vi "AnotherOne.vi"() -> ()   [LabVIEW 2016]
uses:
  <vilib>/DAQmx/write.llb/DAQmx Write (Digital Bool 1Line 1Point).vi
  <vilib>/DAQmx/read.llb/DAQmx Read (Digital Bool 1Line 1Point).vi
  <vilib>/DAQmx/create/channels.llb/DAQmx Create Channel (DI-Digital Input).vi
  <vilib>/DAQmx/create/channels.llb/DAQmx Create Channel (DO-Digital Output).vi
  <vilib>/DAQmx/miscellaneous.llb/DAQmx Fill In Error Info.vi
panel:
  out "Start Button":bool
  out "Stop Button":bool
  out "Bottom Thing":bool
  out "Bottom Solenoid":bool
  in  "Chain Motor":bool
  in  "Sort Solenoid":bool
  in  "Rotary":bool
  in  "Belt motor":bool
  in  "Reject Solenoid":bool
  out "Assembled":bool
  out "Bottom Metal":bool
  out "Dropper Thing":bool
  out "Top Solenoid":bool
  out "Top Thing":bool
  out "Top Metal":bool
  in  "stop":bool
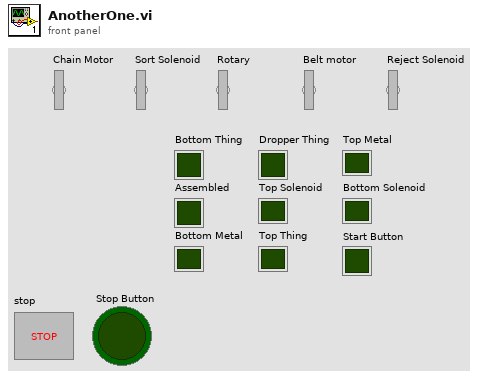
[diagram p1: front panel]
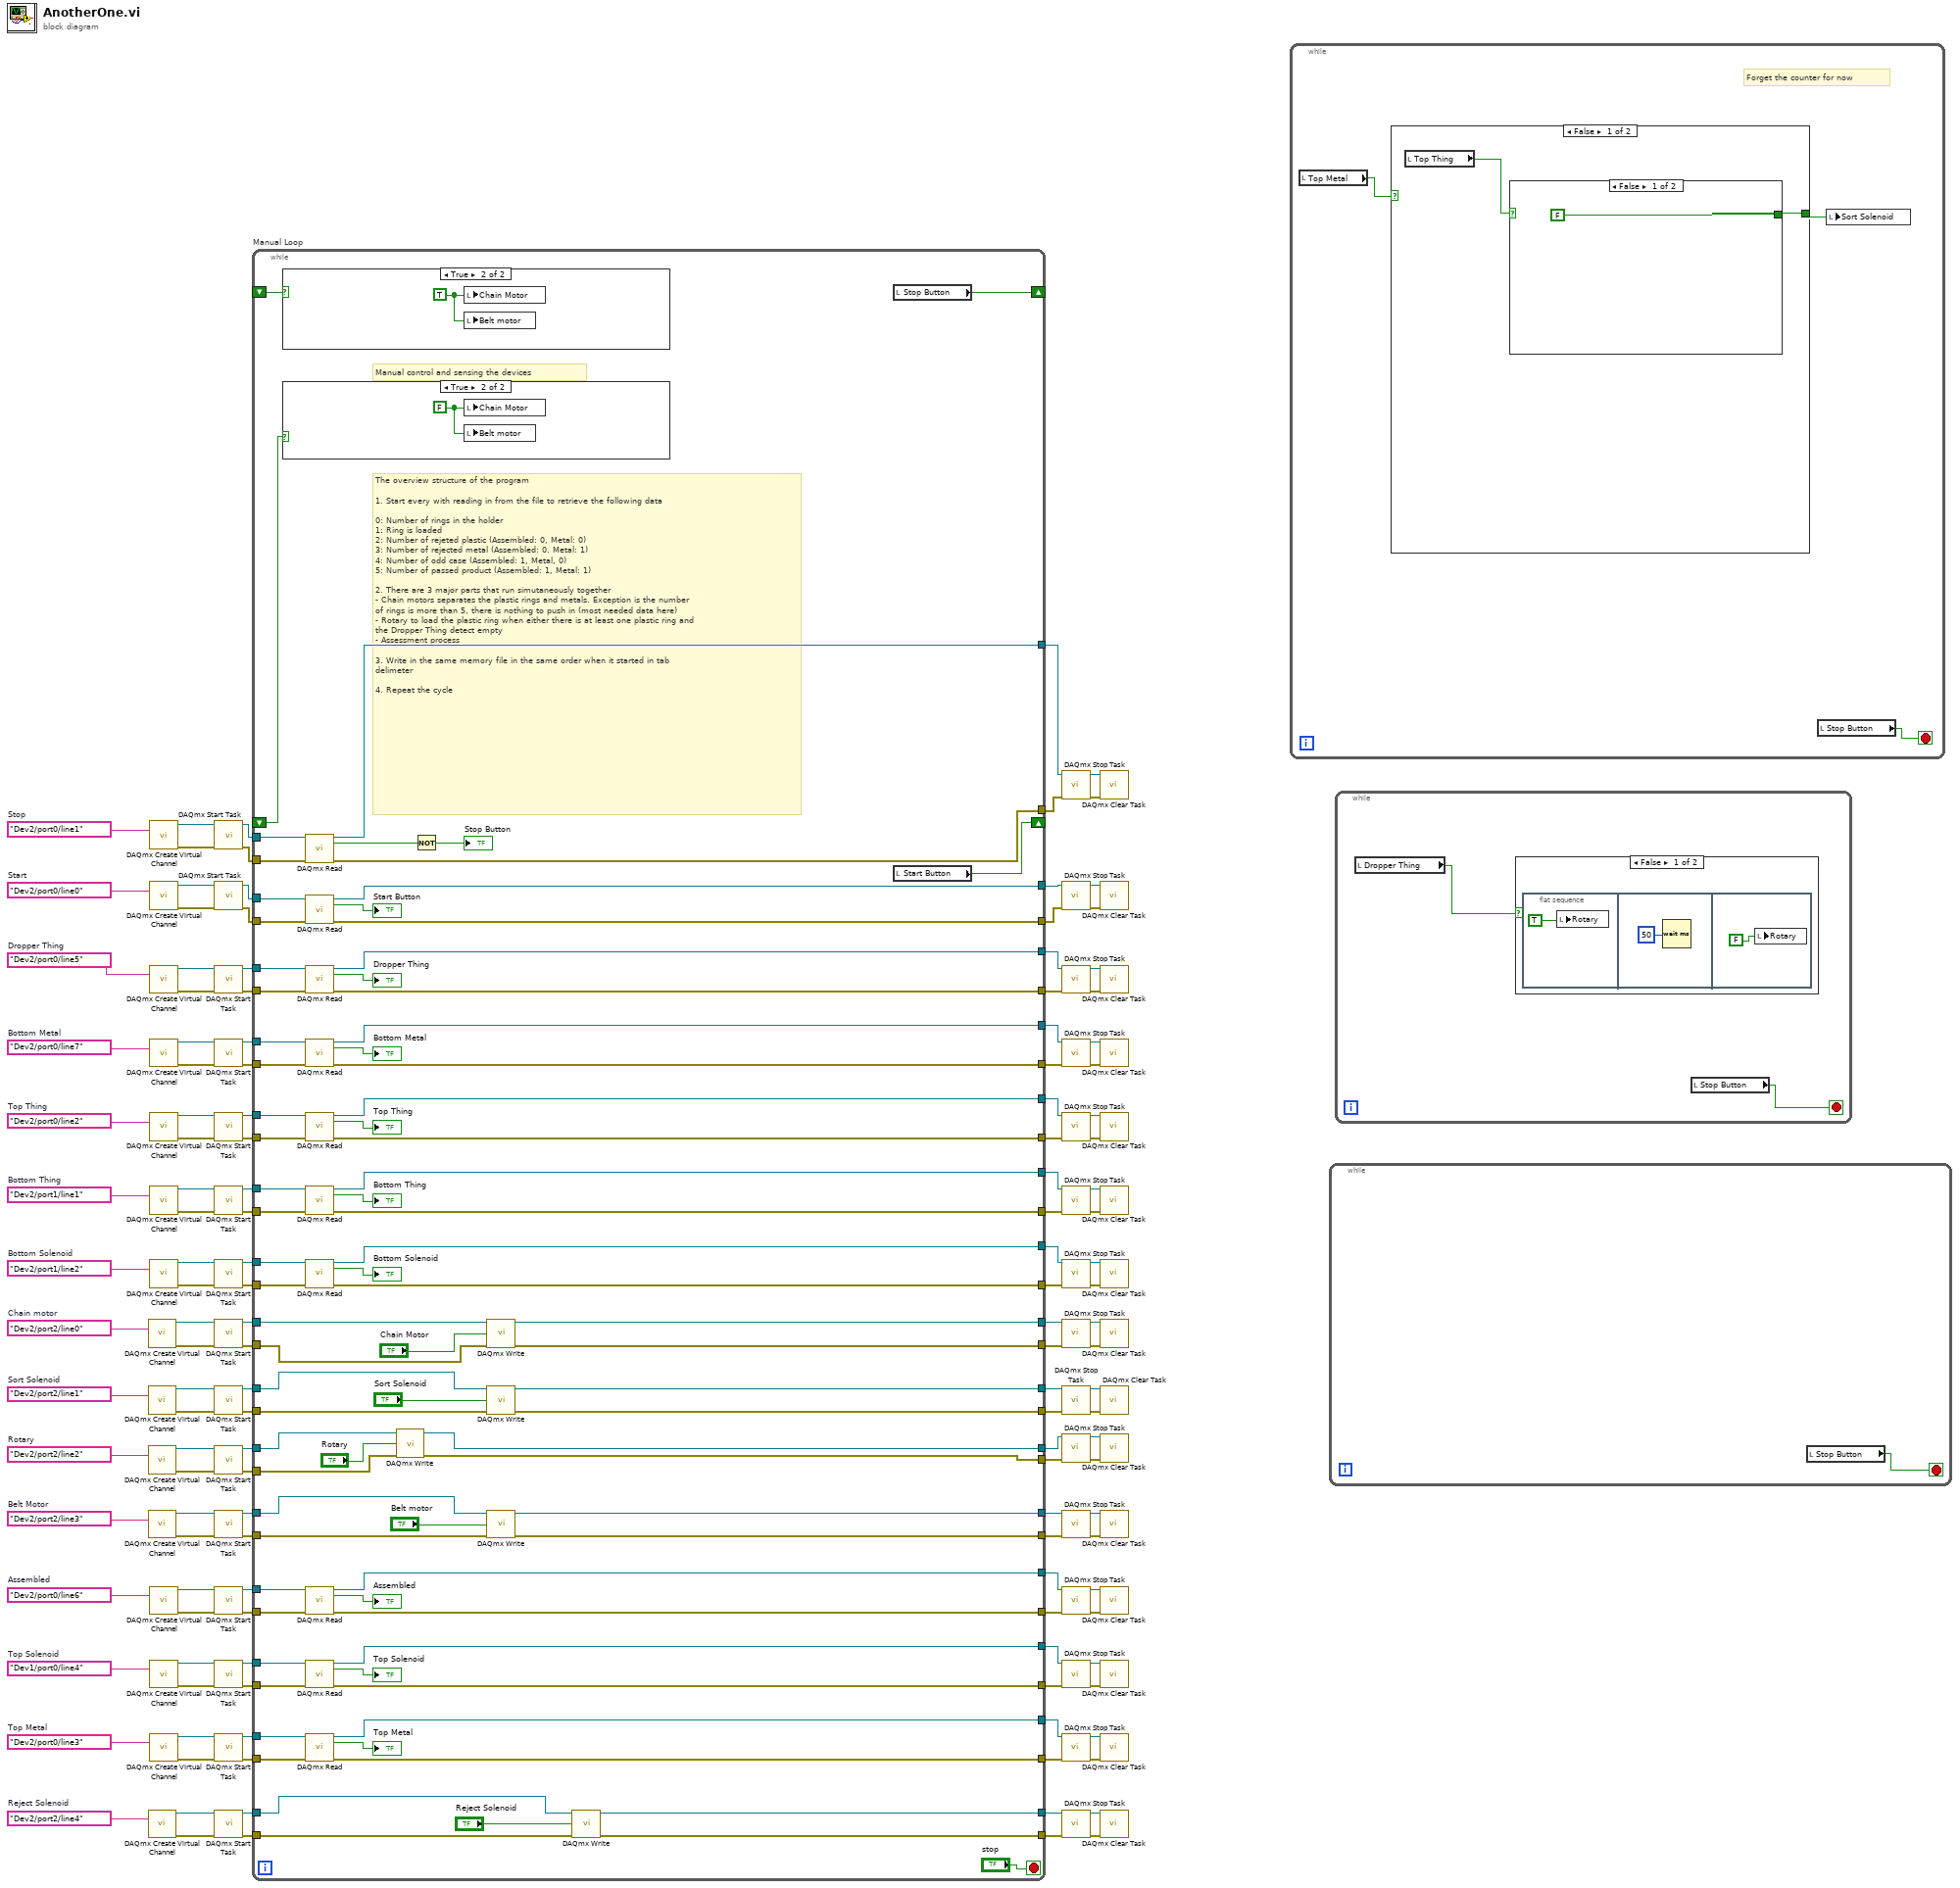
[diagram p0: block diagram]
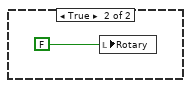
[diagram p2: hidden frame]
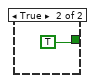
[diagram p3: hidden frame]
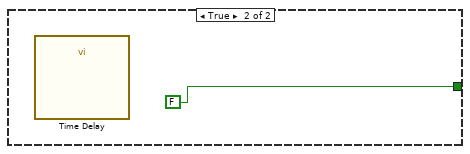
[diagram p4: hidden frame]
diagram:
  w95 = tag "Dev2/port1/line2"  # Bottom Solenoid
  w96 = tag "Dev2/port1/line1"  # Bottom Thing
  w101 = tag "Dev2/port0/line6"  # Assembled
  w102 = tag "Dev2/port0/line7"  # Bottom Metal
  w107 = tag "Dev2/port0/line5"  # Dropper Thing
  w108 = tag "Dev1/port0/line4"  # Top Solenoid
  w113 = tag "Dev2/port0/line3"  # Top Metal
  w114 = tag "Dev2/port0/line2"  # Top Thing
  w117 = tag "Dev2/port2/line4"  # Reject Solenoid
  w122 = tag "Dev2/port2/line3"  # Belt Motor
  w123 = tag "Dev2/port2/line2"  # Rotary
  w132 = tag "Dev2/port2/line1"  # Sort Solenoid
  w133 = tag "Dev2/port2/line0"  # Chain motor
  w134 = tag "Dev2/port0/line1"  # Stop
  w135 = tag "Dev2/port0/line0"  # Start
  n1 = call-poly <vilib>:"DAQmx Create Virtual Channel.vi"("lines"=w133) -> ("task out"=w127:refnum<k21>, "error out"=w126:errorcluster)  [unwired: 13 in]
  n2 = call-poly <vilib>:"DAQmx Create Virtual Channel.vi"("lines"=w132) -> ("task out"=w125:refnum<k21>, "error out"=w124:errorcluster)  [unwired: 13 in]
  n3 = call-poly <vilib>:"DAQmx Create Virtual Channel.vi"("lines"=w123) -> ("task out"=w121:refnum<k21>, "error out"=w120:errorcluster)  [unwired: 13 in]
  n4 = call-poly <vilib>:"DAQmx Create Virtual Channel.vi"("lines"=w122) -> ("task out"=w119:refnum<k21>, "error out"=w118:errorcluster)  [unwired: 13 in]
  n5 = call-poly <vilib>:"DAQmx Create Virtual Channel.vi"("lines"=w117) -> ("task out"=w116:refnum<k21>, "error out"=w115:errorcluster)  [unwired: 13 in]
  n6 = call-poly <vilib>:"DAQmx Create Virtual Channel.vi"("lines"=w134) -> ("task out"=w129:refnum<k21>, "error out"=w128:errorcluster)  [unwired: 13 in]
  n7 = call-poly <vilib>:"DAQmx Create Virtual Channel.vi"("lines"=w135) -> ("task out"=w130:refnum<k21>, "error out"=w131:errorcluster)  [unwired: 13 in]
  n8 = call-poly <vilib>:"DAQmx Create Virtual Channel.vi"("lines"=w107) -> ("task out"=w104:refnum<k21>, "error out"=w103:errorcluster)  [unwired: 13 in]
  n9 = call-poly <vilib>:"DAQmx Create Virtual Channel.vi"("lines"=w102) -> ("task out"=w99:refnum<k21>, "error out"=w100:errorcluster)  [unwired: 13 in]
  n10 = call-poly <vilib>:"DAQmx Create Virtual Channel.vi"("lines"=w114) -> ("task out"=w111:refnum<k21>, "error out"=w112:errorcluster)  [unwired: 13 in]
  n11 = call-poly <vilib>:"DAQmx Create Virtual Channel.vi"("lines"=w96) -> ("task out"=w93:refnum<k21>, "error out"=w94:errorcluster)  [unwired: 13 in]
  n12 = call-poly <vilib>:"DAQmx Create Virtual Channel.vi"("lines"=w95) -> ("task out"=w92:refnum<k21>, "error out"=w91:errorcluster)  [unwired: 13 in]
  n13 = call-poly <vilib>:"DAQmx Create Virtual Channel.vi"("lines"=w101) -> ("task out"=w98:refnum<k21>, "error out"=w97:errorcluster)  [unwired: 13 in]
  n14 = call-poly <vilib>:"DAQmx Create Virtual Channel.vi"("lines"=w108) -> ("task out"=w105:refnum<k21>, "error out"=w106:errorcluster)  [unwired: 13 in]
  n15 = call-poly <vilib>:"DAQmx Create Virtual Channel.vi"("lines"=w113) -> ("task out"=w110:refnum<k21>, "error out"=w109:errorcluster)  [unwired: 13 in]
  n16 = call <vilib>:"DAQmx Start Task.vi"("task/channels in"=w129, "error in"=w128) -> ("task out"=w88:refnum<k21>, "error out"=w87:errorcluster)  [unwired: 12 in]
  n17 = call <vilib>:"DAQmx Start Task.vi"("task/channels in"=w130, "error in"=w131) -> ("task out"=w90:refnum<k21>, "error out"=w89:errorcluster)  [unwired: 12 in]
  n18 = call <vilib>:"DAQmx Start Task.vi"("task/channels in"=w104, "error in"=w103) -> ("task out"=w27:refnum<k21>, "error out"=w28:errorcluster)  [unwired: 12 in]
  n19 = call <vilib>:"DAQmx Start Task.vi"("task/channels in"=w99, "error in"=w100) -> ("task out"=w30:refnum<k21>, "error out"=w29:errorcluster)  [unwired: 12 in]
  n20 = call <vilib>:"DAQmx Start Task.vi"("task/channels in"=w111, "error in"=w112) -> ("task out"=w78:refnum<k21>, "error out"=w77:errorcluster)  [unwired: 12 in]
  n21 = call <vilib>:"DAQmx Start Task.vi"("task/channels in"=w93, "error in"=w94) -> ("task out"=w44:refnum<k21>, "error out"=w43:errorcluster)  [unwired: 12 in]
  n22 = call <vilib>:"DAQmx Start Task.vi"("task/channels in"=w92, "error in"=w91) -> ("task out"=w40:refnum<k21>, "error out"=w39:errorcluster)  [unwired: 12 in]
  n23 = call <vilib>:"DAQmx Start Task.vi"("task/channels in"=w127, "error in"=w126) -> ("task out"=w20:refnum<k21>, "error out"=w19:errorcluster)  [unwired: 12 in]
  n24 = call <vilib>:"DAQmx Start Task.vi"("task/channels in"=w125, "error in"=w124) -> ("task out"=w18:refnum<k21>, "error out"=w17:errorcluster)  [unwired: 12 in]
  n25 = call <vilib>:"DAQmx Start Task.vi"("task/channels in"=w121, "error in"=w120) -> ("task out"=w2:refnum<k21>, "error out"=w1:errorcluster)  [unwired: 12 in]
  n26 = call <vilib>:"DAQmx Start Task.vi"("task/channels in"=w119, "error in"=w118) -> ("task out"=w6:refnum<k21>, "error out"=w5:errorcluster)  [unwired: 12 in]
  n27 = call <vilib>:"DAQmx Start Task.vi"("task/channels in"=w98, "error in"=w97) -> ("task out"=w36:refnum<k21>, "error out"=w35:errorcluster)  [unwired: 12 in]
  n28 = call <vilib>:"DAQmx Start Task.vi"("task/channels in"=w105, "error in"=w106) -> ("task out"=w24:refnum<k21>, "error out"=w23:errorcluster)  [unwired: 12 in]
  n29 = call <vilib>:"DAQmx Start Task.vi"("task/channels in"=w110, "error in"=w109) -> ("task out"=w70:refnum<k21>, "error out"=w69:errorcluster)  [unwired: 12 in]
  n30 = call <vilib>:"DAQmx Start Task.vi"("task/channels in"=w116, "error in"=w115) -> ("task out"=w12:refnum<k21>, "error out"=w11:errorcluster)  [unwired: 12 in]
  n31 = while "Manual Loop" {
    tunnel: w90 -> [w215]
    tunnel: w89 -> [w214]
    tunnel: w88 -> [w213]
    tunnel: w87 -> [w212]
    tunnel: [w211] -> w84
    tunnel: [w210] -> w83
    tunnel: [w209] -> w80
    tunnel: [w208] -> w79
    tunnel: w78 -> [w207]
    tunnel: w77 -> [w206]
    tunnel: [w205] -> w74
    tunnel: [w204] -> w73
    tunnel: w70 -> [w203]
    tunnel: w69 -> [w202]
    tunnel: [w201] -> w68
    tunnel: [w200] -> w67
    tunnel: w44 -> [w199]
    tunnel: w43 -> [w198]
    tunnel: [w197] -> w42
    tunnel: [w196] -> w41
    tunnel: w40 -> [w194]
    tunnel: w39 -> [w193]
    tunnel: [w192] -> w38
    tunnel: [w191] -> w37
    tunnel: w36 -> [w189]
    tunnel: w35 -> [w188]
    tunnel: [w187] -> w34
    tunnel: [w186] -> w33
    tunnel: [w185] -> w32
    tunnel: [w184] -> w31
    tunnel: w30 -> [w183]
    tunnel: w29 -> [w182]
    tunnel: w28 -> [w181]
    tunnel: w27 -> [w180]
    tunnel: [w179] -> w26
    tunnel: [w178] -> w25
    tunnel: w24 -> [w177]
    tunnel: w23 -> [w176]
    tunnel: [w175] -> w22
    tunnel: [w174] -> w21
    tunnel: w20 -> [w173]
    tunnel: w19 -> [w172]
    tunnel: w18 -> [w171]
    tunnel: w17 -> [w170]
    tunnel: [w169] -> w16
    tunnel: [w168] -> w15
    tunnel: [w167] -> w14
    tunnel: [w166] -> w13
    tunnel: w12 -> [w165]
    tunnel: w11 -> [w164]
    tunnel: [w163] -> w10
    tunnel: [w162] -> w9
    tunnel: [w161] -> w8
    tunnel: [w160] -> w7
    tunnel: w6 -> [w159]
    tunnel: w5 -> [w158]
    tunnel: [w157] -> w4
    tunnel: [w156] -> w3
    tunnel: w2 -> [w155]
    tunnel: w1 -> [w154]
    shift-right: [w148] -> _
    shift-left: _ -> [w142]
    shift-right: [w147] -> _
    shift-left: _ -> [w143]
    stop <- "stop" stop-if-true
    # "The overview structure of the program\n\n1. Start every with reading in from the file to retrieve the following data\n\n0: Number of rings in the holder\n1: Ring is loaded\n2: Number of rejeted plastic (Assembled: 0, Metal: 0)\n3: Number of rejected metal (Assembled: 0. Metal: 1)\n4: Number of odd case (Assembled: 1, Metal, 0)\n5: Number of passed product (Assembled: 1, Metal: 1)\n\n2. There are 3 major parts that run simutaneously together\n- Chain motors separates the plastic rings and metals. Exception is the number\nof rings is more than 5, there is nothing to push in (most needed data here)\n- Rotary to load the plastic ring when either there is at least one plastic ring and\nthe Dropper Thing detect empty\n- Assessment process\n\n3. Write in the same memory file in the same order when it started in tab\ndelimeter\n\n4. Repeat the cycle"
    # "Manual control and sensing the devices"
    n32 = case shown="True" w143 {
      frame False {
      }
      frame True {
        w218 = TRUE
        n33 = local write "Chain Motor"(w218) -> ()
        n34 = local write "Belt motor"(w218) -> ()
      }
    }
    n35 = case shown="True" w142 {
      frame False {
      }
      frame True {
        w217 = FALSE
        n36 = local write "Chain Motor"(w217) -> ()
        n37 = local write "Belt motor"(w217) -> ()
      }
    }
    n38 = call-poly <vilib>:"DAQmx Read.vi"("task/channels in"=w213, "error in"=w212) -> ("task out"=w211:refnum<k21>, "data"=w136:bool, "error out"=w210:errorcluster)  [unwired: 11 in]
    n39 = call-poly <vilib>:"DAQmx Read.vi"("task/channels in"=w215, "error in"=w214) -> ("task out"=w209:refnum<k21>, "data"=→"Start Button":bool, "error out"=w208:errorcluster)  [unwired: 11 in]
    n40 = call-poly <vilib>:"DAQmx Read.vi"("task/channels in"=w180, "error in"=w181) -> ("task out"=w179:refnum<k21>, "data"=→"Dropper Thing":bool, "error out"=w178:errorcluster)  [unwired: 11 in]
    n41 = call-poly <vilib>:"DAQmx Read.vi"("task/channels in"=w183, "error in"=w182) -> ("task out"=w185:refnum<k21>, "data"=→"Bottom Metal":bool, "error out"=w184:errorcluster)  [unwired: 11 in]
    n42 = call-poly <vilib>:"DAQmx Read.vi"("task/channels in"=w207, "error in"=w206) -> ("task out"=w204:refnum<k21>, "data"=→"Top Thing":bool, "error out"=w205:errorcluster)  [unwired: 11 in]
    n43 = call-poly <vilib>:"DAQmx Read.vi"("task/channels in"=w199, "error in"=w198) -> ("task out"=w197:refnum<k21>, "data"=→"Bottom Thing":bool, "error out"=w196:errorcluster)  [unwired: 11 in]
    n44 = call-poly <vilib>:"DAQmx Read.vi"("task/channels in"=w194, "error in"=w193) -> ("task out"=w192:refnum<k21>, "data"=→"Bottom Solenoid":bool, "error out"=w191:errorcluster)  [unwired: 11 in]
    n45 = call-poly <vilib>:"DAQmx Read.vi"("task/channels in"=w189, "error in"=w188) -> ("task out"=w187:refnum<k21>, "data"=→"Assembled":bool, "error out"=w186:errorcluster)  [unwired: 11 in]
    n46 = call-poly <vilib>:"DAQmx Read.vi"("task/channels in"=w177, "error in"=w176) -> ("task out"=w175:refnum<k21>, "data"=→"Top Solenoid":bool, "error out"=w174:errorcluster)  [unwired: 11 in]
    n47 = call-poly <vilib>:"DAQmx Read.vi"("task/channels in"=w203, "error in"=w202) -> ("task out"=w201:refnum<k21>, "data"=→"Top Metal":bool, "error out"=w200:errorcluster)  [unwired: 11 in]
    n48 = call-poly <vilib>:"DAQmx Write.vi"("task/channels in"=w155, "data"="Rotary", "error in"=w154) -> ("task out"=w156:refnum<k21>, "error out"=w157:errorcluster)  [unwired: 10 in, 1 out]
    n49 = Not(x=w136) -> (.not. x?=→"Stop Button":bool)
    n50 = call-poly <vilib>:"DAQmx Write.vi"("task/channels in"=w173, "data"="Chain Motor", "error in"=w172) -> ("task out"=w169:refnum<k21>, "error out"=w168:errorcluster)  [unwired: 10 in, 1 out]
    n51 = call-poly <vilib>:"DAQmx Write.vi"("task/channels in"=w171, "data"="Sort Solenoid", "error in"=w170) -> ("task out"=w167:refnum<k21>, "error out"=w166:errorcluster)  [unwired: 10 in, 1 out]
    n52 = call-poly <vilib>:"DAQmx Write.vi"("task/channels in"=w159, "data"="Belt motor", "error in"=w158) -> ("task out"=w161:refnum<k21>, "error out"=w160:errorcluster)  [unwired: 10 in, 1 out]
    n53 = call-poly <vilib>:"DAQmx Write.vi"("task/channels in"=w165, "data"="Reject Solenoid", "error in"=w164) -> ("task out"=w163:refnum<k21>, "error out"=w162:errorcluster)  [unwired: 10 in, 1 out]
    n54 = local read "Stop Button"() -> (w147:bool)
    n55 = local read "Start Button"() -> (w148:bool)
  }
  n56 = call <vilib>:"DAQmx Stop Task.vi"("task/channels in"=w84, "error in"=w83) -> ("task out"=w85:refnum<k21>, "error out"=w86:errorcluster)  [unwired: 12 in]
  n57 = call <vilib>:"DAQmx Stop Task.vi"("task/channels in"=w80, "error in"=w79) -> ("task out"=w81:refnum<k21>, "error out"=w82:errorcluster)  [unwired: 12 in]
  n58 = call <vilib>:"DAQmx Stop Task.vi"("task/channels in"=w26, "error in"=w25) -> ("task out"=w55:refnum<k21>, "error out"=w56:errorcluster)  [unwired: 12 in]
  n59 = call <vilib>:"DAQmx Stop Task.vi"("task/channels in"=w32, "error in"=w31) -> ("task out"=w53:refnum<k21>, "error out"=w54:errorcluster)  [unwired: 12 in]
  n60 = call <vilib>:"DAQmx Stop Task.vi"("task/channels in"=w73, "error in"=w74) -> ("task out"=w75:refnum<k21>, "error out"=w76:errorcluster)  [unwired: 12 in]
  n61 = call <vilib>:"DAQmx Stop Task.vi"("task/channels in"=w42, "error in"=w41) -> ("task out"=w65:refnum<k21>, "error out"=w66:errorcluster)  [unwired: 12 in]
  n62 = call <vilib>:"DAQmx Stop Task.vi"("task/channels in"=w38, "error in"=w37) -> ("task out"=w63:refnum<k21>, "error out"=w64:errorcluster)  [unwired: 12 in]
  n63 = call <vilib>:"DAQmx Stop Task.vi"("task/channels in"=w16, "error in"=w15) -> ("task out"=w61:refnum<k21>, "error out"=w62:errorcluster)  [unwired: 12 in]
  n64 = call <vilib>:"DAQmx Stop Task.vi"("task/channels in"=w14, "error in"=w13) -> ("task out"=w59:refnum<k21>, "error out"=w60:errorcluster)  [unwired: 12 in]
  n65 = call <vilib>:"DAQmx Stop Task.vi"("task/channels in"=w3, "error in"=w4) -> ("task out"=w49:refnum<k21>, "error out"=w50:errorcluster)  [unwired: 12 in]
  n66 = call <vilib>:"DAQmx Stop Task.vi"("task/channels in"=w8, "error in"=w7) -> ("task out"=w47:refnum<k21>, "error out"=w48:errorcluster)  [unwired: 12 in]
  n67 = call <vilib>:"DAQmx Stop Task.vi"("task/channels in"=w34, "error in"=w33) -> ("task out"=w51:refnum<k21>, "error out"=w52:errorcluster)  [unwired: 12 in]
  n68 = call <vilib>:"DAQmx Stop Task.vi"("task/channels in"=w22, "error in"=w21) -> ("task out"=w57:refnum<k21>, "error out"=w58:errorcluster)  [unwired: 12 in]
  n69 = call <vilib>:"DAQmx Stop Task.vi"("task/channels in"=w68, "error in"=w67) -> ("task out"=w71:refnum<k21>, "error out"=w72:errorcluster)  [unwired: 12 in]
  n70 = call <vilib>:"DAQmx Stop Task.vi"("task/channels in"=w10, "error in"=w9) -> ("task out"=w45:refnum<k21>, "error out"=w46:errorcluster)  [unwired: 12 in]
  n71 = call <vilib>:"DAQmx Clear Task.vi"("task in"=w85, "error in"=w86) -> ()  [unwired: 13 in, 1 out]
  n72 = call <vilib>:"DAQmx Clear Task.vi"("task in"=w81, "error in"=w82) -> ()  [unwired: 13 in, 1 out]
  n73 = call <vilib>:"DAQmx Clear Task.vi"("task in"=w55, "error in"=w56) -> ()  [unwired: 13 in, 1 out]
  n74 = call <vilib>:"DAQmx Clear Task.vi"("task in"=w53, "error in"=w54) -> ()  [unwired: 13 in, 1 out]
  n75 = call <vilib>:"DAQmx Clear Task.vi"("task in"=w75, "error in"=w76) -> ()  [unwired: 13 in, 1 out]
  n76 = call <vilib>:"DAQmx Clear Task.vi"("task in"=w65, "error in"=w66) -> ()  [unwired: 13 in, 1 out]
  n77 = call <vilib>:"DAQmx Clear Task.vi"("task in"=w63, "error in"=w64) -> ()  [unwired: 13 in, 1 out]
  n78 = call <vilib>:"DAQmx Clear Task.vi"("task in"=w61, "error in"=w62) -> ()  [unwired: 13 in, 1 out]
  n79 = call <vilib>:"DAQmx Clear Task.vi"("task in"=w59, "error in"=w60) -> ()  [unwired: 13 in, 1 out]
  n80 = call <vilib>:"DAQmx Clear Task.vi"("task in"=w49, "error in"=w50) -> ()  [unwired: 13 in, 1 out]
  n81 = call <vilib>:"DAQmx Clear Task.vi"("task in"=w47, "error in"=w48) -> ()  [unwired: 13 in, 1 out]
  n82 = call <vilib>:"DAQmx Clear Task.vi"("task in"=w51, "error in"=w52) -> ()  [unwired: 13 in, 1 out]
  n83 = call <vilib>:"DAQmx Clear Task.vi"("task in"=w57, "error in"=w58) -> ()  [unwired: 13 in, 1 out]
  n84 = call <vilib>:"DAQmx Clear Task.vi"("task in"=w71, "error in"=w72) -> ()  [unwired: 13 in, 1 out]
  n85 = call <vilib>:"DAQmx Clear Task.vi"("task in"=w45, "error in"=w46) -> ()  [unwired: 13 in, 1 out]
  n86 = while {
    stop <- w220 stop-if-true
    # "Forget the counter for now"
    n87 = local read "Top Metal"() -> (w221:bool)
    n88 = case shown="False" w221 {
      tunnel: [w223 FALSE] -> w219
      frame False {
        n89 = local read "Top Thing"() -> (w222:bool)
        n90 = case shown="False" w222 {
          tunnel: [FALSE TRUE] -> w223
          frame False {
          }
          frame True {
          }
        }
      }
      frame True {
        n91 = call "Time Delay"() -> ()  [unwired: 11 in, 1 out]
      }
    }
    n92 = local read "Stop Button"() -> (w220:bool)
    n93 = local write "Sort Solenoid"(w219) -> ()
  }
  n94 = while {
    stop <- w227 stop-if-true
    n95 = local read "Stop Button"() -> (w227:bool)
  }
  n96 = while {
    stop <- w229 stop-if-true
    n97 = local read "Dropper Thing"() -> (w228:bool)
    n98 = case shown="False" w228 {
      frame False {
        n99 = flat-sequence {
          frame #0 {
            n100 = local write "Rotary"(TRUE) -> ()
          }
          frame #1 {
            n101 = Wait (ms)(milliseconds to wait=u32 50) -> ()  [unwired: 1 out]
          }
          frame #2 {
            n102 = local write "Rotary"(FALSE) -> ()
          }
        }
      }
      frame True {
        n103 = local write "Rotary"(FALSE) -> ()
      }
    }
    n104 = local read "Stop Button"() -> (w229:bool)
  }
